vi "VM3 - 2D Array of DBL.vi"(5 "cmd (read)":enum16{"create", "destroy", "write", "read"}(ring)=enum."read", 7 "VC Handle":T2, 8 "error in":errorcluster, 9 "writer ID":u32, 10 "value in":dbl[][](array[numeric]), 11 "name_spec":string) -> (0 "error out":errorcluster, 1 "stats":T1, 2 "value out":dbl[][](array[numeric]), 3 "dup name_spec":string)   [LabVIEW 2021]
doc: "This VI manages variables of the <b>2D Array of DBL</b> data type. Refer to the VI Help for more details.\n\n<b>cmd (read)</b> specifies the operation to perform on the variable: create, write, read, or destroy.\n\n<b>VC Handle</b> specifies the handle of the variable context. To operate on a global variable, pass -1 to this input. <b>name_spec</b> is the name specifier of the desired variable; usually, it is merely a variable name (see the VI Help for more options).\n\n<b>value in</b> and <b>value out</b> are the input and output values written to or read from the variable, respectively.\n\n<b>writer ID</b> specifies the Writer ID to be set along with the new value when writing or creating a variable.\n\n<b>stats</b> returns information about the most recent value of the variable, such as its Writer ID, update time, and update counter.\n\n::: CalcExpress Toolkit :::\nCopyright (c) 2000-2026 Konstantin Shifershteyn. All rights reserved."
uses:
  cetypes.llb/VarMan Variable Context Handle.ctl
  cetypes.llb/VarMan Variable Data Statistics.ctl
  cetypes.llb/VarMan Error Code.ctl
  cersrc/celveng32.dll
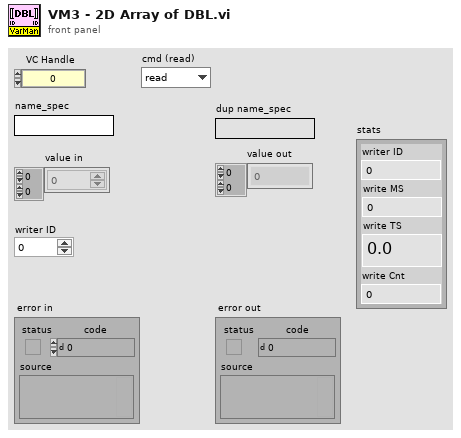
[diagram p1: front panel]
types:
  T1 = typedef "VarMan Variable Data Statistics.ctl" = cluster{"writer ID":u32, "write MS":u32, "write TS":dbl, "write Cnt":u32}
  T2 = typedef "VarMan Variable Context Handle.ctl" = i32
  T3 = enum32{"String", "DBL Number", "identifier", "1D Array of DBL", "2D Array of DBL", "CDB Number", "1D Array of CDB", "2D Array of CDB", "1D Array of String", "2D Array of String", "Unknown data type"}
  T4 = typedef "VarMan Error Code.ctl" = u16
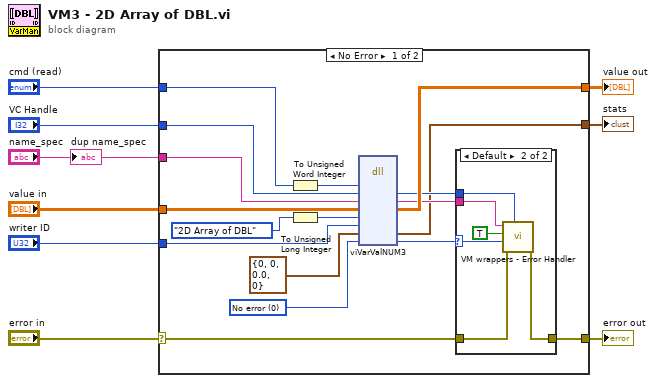
[diagram p0: block diagram]
diagram:
  n1 = case shown="No Error" "error in" {
    selector: "error in" -> [w14 w35]
    tunnel: [w26 w35] -> w3
    tunnel: "value in" -> [w24 w34]
    tunnel: "name_spec" -> [w23 _]
    tunnel: "VC Handle" -> [w22 _]
    tunnel: [w21 w34] -> w2
    tunnel: "cmd (read)" -> [w20 _]
    tunnel: "writer ID" -> [w12 _]
    tunnel: [w10 _] -> w1
    frame No Error {
      w19 = T4 0 items=["No error", "Invalid variable type", "Variable not found", "Variable already exists", "Invalid context handle", "Input error", "Invalid data format", "No history attached", "History already attached", "Invalid history parameters", "Wrong variable name", "Wrong alias name", "Non-unique alias", "Alias not found", "No alias associated", "Alias already associated", "Wrong context name", "Non-unique context name", "Context name not found", "Invalid parameter", "Generic error", "Memory Full", "Unrecognized LV error", "Unknown error code"] ("err code")
      n2 = To Unsigned Word Integer(number=w20) -> (unsigned 16bit integer=w15:u16)
      n3 = To Unsigned Long Integer(number=T3."2D Array of DBL" ("data type")) -> (unsigned 32bit integer=w13:u32)
      n4 = dll-call lib="C:/LV Projects/CalcExpress 40 LV2021/vi.lib/addons/CalcExpress/cersrc/celveng*.dll" fn="viVarValNUM3"("cmd"=w15, "vch"=w22, "name"=w23, "val"=w24, "type"=w13, "writerID"=w12, "wrStats"=T1 {"writer ID"=0, "write MS"=0, "write TS"=0.0, "write Cnt"=0} ("stats"), "errc"=w19) -> ("vch"=w16:i32, "name"=w17:string, "val"=w21:dbl[][], "wrStats"=w10:T1, "errc"=w18:T4)  [unwired: 7 in, 2 out]
      n5 = case shown="Default" w18 {
        selector: w18 -> [_ w30]
        tunnel: [w27 w33] -> w26
        tunnel: w14 -> [w27 w32]
        tunnel: w17 -> [_ w29]
        tunnel: w16 -> [_ w28]
        frame 0 {
        }
        frame Default {
          n6 = call "VM wrappers - Error Handler.vi"("VC Handle"=w28, "error before"=w32, "VarMan error"=w30, "show name spec (F)"=TRUE, "name spec"=w29) -> ("error out"=w33:errorcluster)  [unwired: 5 in, 1 out]
        }
      }
    }
    frame Error {
    }
  }
  "value out" <- w2
  "error out" <- w3
  "stats" <- w1
  "dup name_spec" <- "name_spec"
